vi "Connect.vi"(8 "error in (no error)":errorcluster, 11 "object in":refnum<class "Type_Channel.lvclass">) -> (0 "error out":errorcluster, 2 "Success?":bool, 3 "object out":refnum<class "Type_Channel.lvclass">)   [LabVIEW 2021, in "Template-ChannelsChild.lvlib" / "Type_Channel.lvclass"]
uses:
  Type_Channel.lvclass
  Type_Channel.lvclass/Type_Channel.ctl
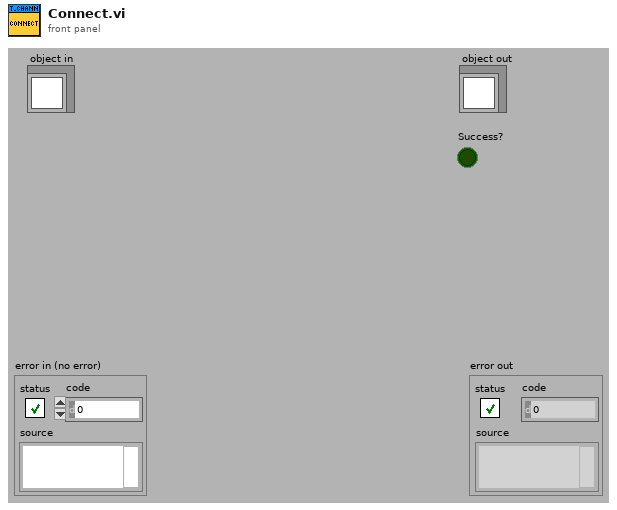
[diagram p1: front panel]
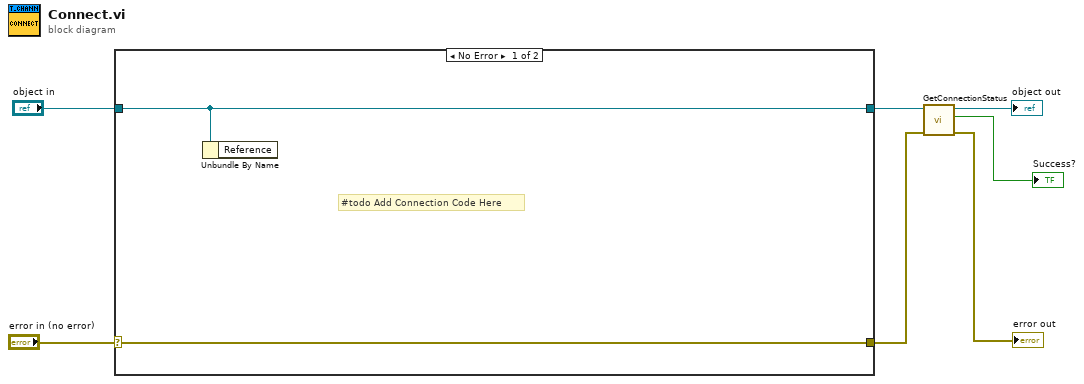
[diagram p0: block diagram]
diagram:
  n1 = case shown="No Error" "error in (no error)" {
    selector: "error in (no error)" -> [w9 w11]
    tunnel: [w9 w11] -> w3
    tunnel: [w8 w10] -> w5
    tunnel: "object in" -> [w8 w10]
    frame No Error {
      # "#todo Add Connection Code Here"
      n2 = Unbundle By Name(w8) -> ()  [unwired: 1 out]
    }
    frame Error {
    }
  }
  n3 = call-dynamic "GetConnectionStatus.vi"("error in (no error)"=w3, "object in"=w5) -> ("error out"=→"error out":errorcluster, "Connected?"=→"Success?":bool, "object out"=→"object out":refnum<class "Type_Channel.lvclass">)  [unwired: 7 in]
